vi "Find Method.vi"(8 "error in (no error)":errorcluster, 10 "Method Name":string, 11 "Declaring Type in":refnum<k24>) -> (0 "error out":errorcluster, 2 "Method Info":refnum<k24>, 3 "Declaring Type out":refnum<k24>)   [LabVIEW 2026, in "ToastNotification.lvlib" / "Reflection DotNet.lvlib"]
doc: "Native System.Type.GetMethod call. Borrow Declaring Type in and acquire Method Info for Method Name. This overload resolves by name and can report an ambiguous match for overloaded methods. Declaring Type out is an alias. Caller closes the acquired MethodInfo."
uses:
  Reflection DotNet.lvlib
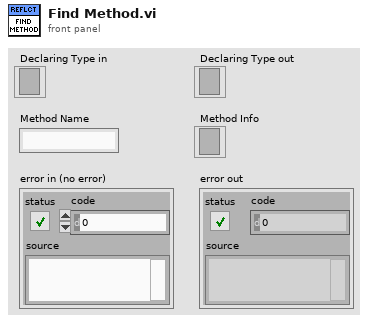
[diagram p1: front panel]
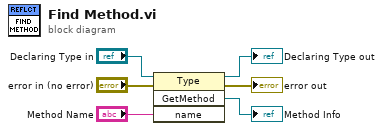
[diagram p0: block diagram]
diagram:
  n1 = invoke class="Type" method="GetMethod"(reference="Declaring Type in", error in="error in (no error)", "name"="Method Name") -> (reference out=→"Declaring Type out":refnum<k24>, error out=→"error out":errorcluster, "GetMethod"=→"Method Info":refnum<k24>)  [unwired: 1 in, 1 out]
